vi "csb hdlc state size.vi"(8 "error in (no error)":errorcluster) -> (0 "error out":errorcluster, 3 "function return":i32)   [LabVIEW 2021, in "CANsub_Codec.lvlib"]
doc: "int32_t csb_hdlc_state_size(void);"
uses:
  CANsub_Codec.lvlib
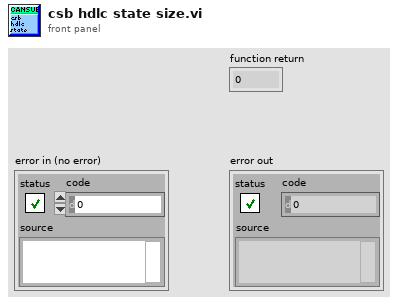
[diagram p1: front panel]
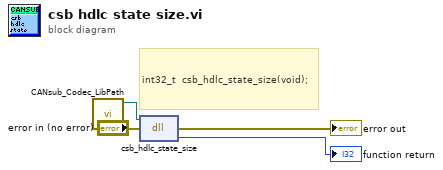
[diagram p0: block diagram]
diagram:
  # "int32_t  csb_hdlc_state_size(void);"
  n1 = call "CANsub_Codec_LibPath.vi"() -> ("Path"=w1:path)  [unwired: 11 in]
  n2 = dll-call lib="libcansub_codec.*" fn="csb_hdlc_state_size"(path in=w1, error in="error in (no error)") -> (error out=→"error out":errorcluster, "return type"=→"function return":i32)  [unwired: 1 in, 1 out]
